vi "ECS-GDI-Host.vi"() -> ()   [LabVIEW 2015]
uses:
  <vilib>/addons/Software Calibration Management/XControls/SubHost.xctl
  <vilib>/addons/Software Calibration Management/XControls/SubHost List.xctl
  Typedefs/EPT/Engine Status.ctl
  <vilib>/addons/Software Calibration Management/XControls/TBL1D.xctl
  <vilib>/addons/Software Calibration Management/XControls/Faults.xctl
  ECS-Host.lvlib
  ECS-Shared.lvlib
panel:
  out "CalPointData":sgl[](array[numeric])
  in  "_Refresh":bool
  in  "EngineSpeed_MaxNC":sgl
  in  "EngineSpeed_MaxCrit":sgl
  out "5VPSU_CriticalFault":bool
  out "12VPSU_CriticalFault":bool
  out "BattV_CriticalFault":bool
  in  "_Main Tabs":T1(tab)
  in  "PowerEnable":bool caption="Power Enable"
  out "EngineSpeedFPGA1":sgl(knob) scale=0.0..1000.0 scale format="%#_6p"
  in  "SyncEnable":bool caption="Sync Enable"
  out "ReceivingPrimaryFPGA1":bool caption="Rcvg Primary"
  out "SyncFPGA1":bool caption="Sync"
  out "_BattVPresent":bool caption="Battery"
  out "_12VPresent":bool caption="12V"
  out "_5VPresent":bool caption="5V"
  out "Engine Time":sgl caption="[hr]" format="%0#5_4f"
  out "Time Since Start":sgl caption="[sec]" format="%05.0f"
  in  "Engine Time Reset":bool
  out "_Engine Speed":sgl format="%#.0f"
  out "Software Version":string caption="Version:"
  out "_Engine Status":T2 caption="Engine Status"
  in  "Faults Table":T4(xcontrol)
  in  "_SubHost Tab":T5(tab)
  in  "XNET CAN":T6(xcontrol)
  in  "Power":T6(xcontrol)
  in  "TDK High Voltage Supply":T6(xcontrol)
  in  "NI 9754-1 (ESTTL)":T6(xcontrol)
  in  "NI 9411-1 (Digital Input)":T6(xcontrol)
  in  "NI 9758-2 (PFI/LS)":T6(xcontrol)
  in  "NI 9751-4 (DI Driver)":T6(xcontrol)
  in  "NI 9751-3 (DI Driver)":T6(xcontrol)
  in  "NI 9751-2 (DI Driver)":T6(xcontrol)
  in  "NI 9752-1 (ADCombo)":T6(xcontrol)
  in  "NI 9757-1 (O2)":T6(xcontrol)
  in  "NI 9755-1 (NOx)":T6(xcontrol)
  in  "NI 9759-1 (Throttle)":T6(xcontrol)
  in  "NI 9758-1 (PFI/LS)":T6(xcontrol)
  in  "NI 9751-1 (DI Driver)":T6(xcontrol)
  in  "EPTx":T6(xcontrol)
  in  "Boost Actuation":T6(xcontrol)
  in  "Boost Actuation":T6(xcontrol)
  in  "MPCR":T6(xcontrol)
  in  "VVA Actuation":T6(xcontrol)
  in  "Direct Injectors":T6(xcontrol)
  in  "Engine Specs":T6(xcontrol)
  in  "Sensors":T6(xcontrol)
  in  "Faults":T6(xcontrol) caption="0"
  in  "Rail Pressure Setpoint":T6(xcontrol) caption="1"
  in  "Wastegate Control":T6(xcontrol) caption="1"
  in  "Turbo BPV Control":T6(xcontrol) caption="1"
  in  "Throttle Setpoint":T6(xcontrol) caption="1"
  in  "VVA Setpoint":T6(xcontrol) caption="1"
  in  "Intake Air Desired MAP":T6(xcontrol) caption="0"
  in  "Lambda Command":T6(xcontrol) caption="0"
  in  "Spark Control":T6(xcontrol) caption="1"
  in  "Cranking":T6(xcontrol) caption="0"
  in  "Direct Injection Strategy":T6(xcontrol) caption="2"
  in  "Fuel Quantity":T6(xcontrol) caption="1"
  in  "Load Command":T6(xcontrol) caption="0"
  in  "Intake Air Measured":T6(xcontrol) caption="1"
  in  "Execution Info":T6(xcontrol)
  in  "Calscope and Trends":T6(xcontrol)
  in  "MAP_ManE":bool
  in  "Pedal_ManE":bool
  in  "MEP_ManE":bool
  in  "RailP_ManE":bool
  in  "Pedal_Man":sgl(slide) caption="[bar]" scale=0.0..100.0 scale format="%#4.1f"
  in  "MEP_Man":sgl(slide) caption="[bar]" scale=0.0..25.0 scale format="%#4.1f"
  in  "RailP_Man":sgl(slide) caption="[bar]" scale=0.0..2000.0 scale format="%#4.1f"
  in  "MAP_Man":sgl(slide) caption="[kPa]" scale=0.0..400.0 scale format="%#4.1f"
  in  "ForceSafeState":bool caption="Push to Force Safe State"
  out "Non-Critical Fault":bool
  out "Critical Fault":bool
  in  "ESTOP":bool caption="Push to Stop"
  in  "System":T7(xcontrol)
  in  "Control":T7(xcontrol)
  in  "Engine":T7(xcontrol)
  in  "Hardware":T7(xcontrol)
  in  "_HiddenControls":enum32{"Page 1"}(tab)
  out "RailP_Des":sgl
  out "MAP_Des":sgl
  in  "NominalMEP_Tbl":cluster{"X":sgl[], "Y":sgl[]}(xcontrol)
  out "MEP_Des":sgl caption="EngineLoad_Des"
  out "Pedal_Des":sgl
  out "EngineStatus":u8
  in  "_Default Colors":bool caption="Default Colors"
  in  "_HiddenControls2":enum32{"Page 1"}(tab)
  in  "_VisiblePlots":bool[](array[boolean])
  in  "N Items":u8
  in  "_Signal Units":string[](array[string])
  in  "Colors":sgl[](array[numeric])
  in  "SliderMin":sgl[](array[numeric])
  in  "SliderMax":sgl[](array[numeric])
  out "Units":string
  in  "_Signal Names":string[](array[string])
  in  "CalPointIDs":sgl[](array[numeric])
  out "NamesLong":string
  out "_Chart":T8(graph)
  in  "_Down":bool
  in  "_Up":bool
  in  "_PlotHidden":bool caption="Hide"
  in  "_Delete":bool
  in  "_Add":bool
  out "_Data":string[](array[string])
  in  "_Slider Max":sgl caption="Max"
  in  "_Slider Min":sgl caption="Min"
  in  "_CalpointIDSelect":u16(ring) caption="Signal Name"
  in  "_Color":u32(colorbox)=16777222 caption="Color"
  in  "_Table":i32(listbox)
  in  "_Chart History1":i32=20 caption="Chart History"
  out "_LoadTracking":cluster{"X Buffer":sgl[], "Y Buffer":sgl[]}[](graph) caption="Load Tracking"
  in  "_Chart History2":i32=20 caption="Chart History"
  in  "_Normalize":bool=TRUE caption="Normalize"
  in  "_Var Select":u16(ring) caption="Signal Selection"
  out "_ReturnMap":cluster{"X Buffer":sgl[], "Y Buffer":sgl[]}[](graph) caption="Return Map"
  # "Engine Control System"
  # "RPM"
  # "Customize UI Here"
  # "Customize UI Here"
  # "Customize UI Here"
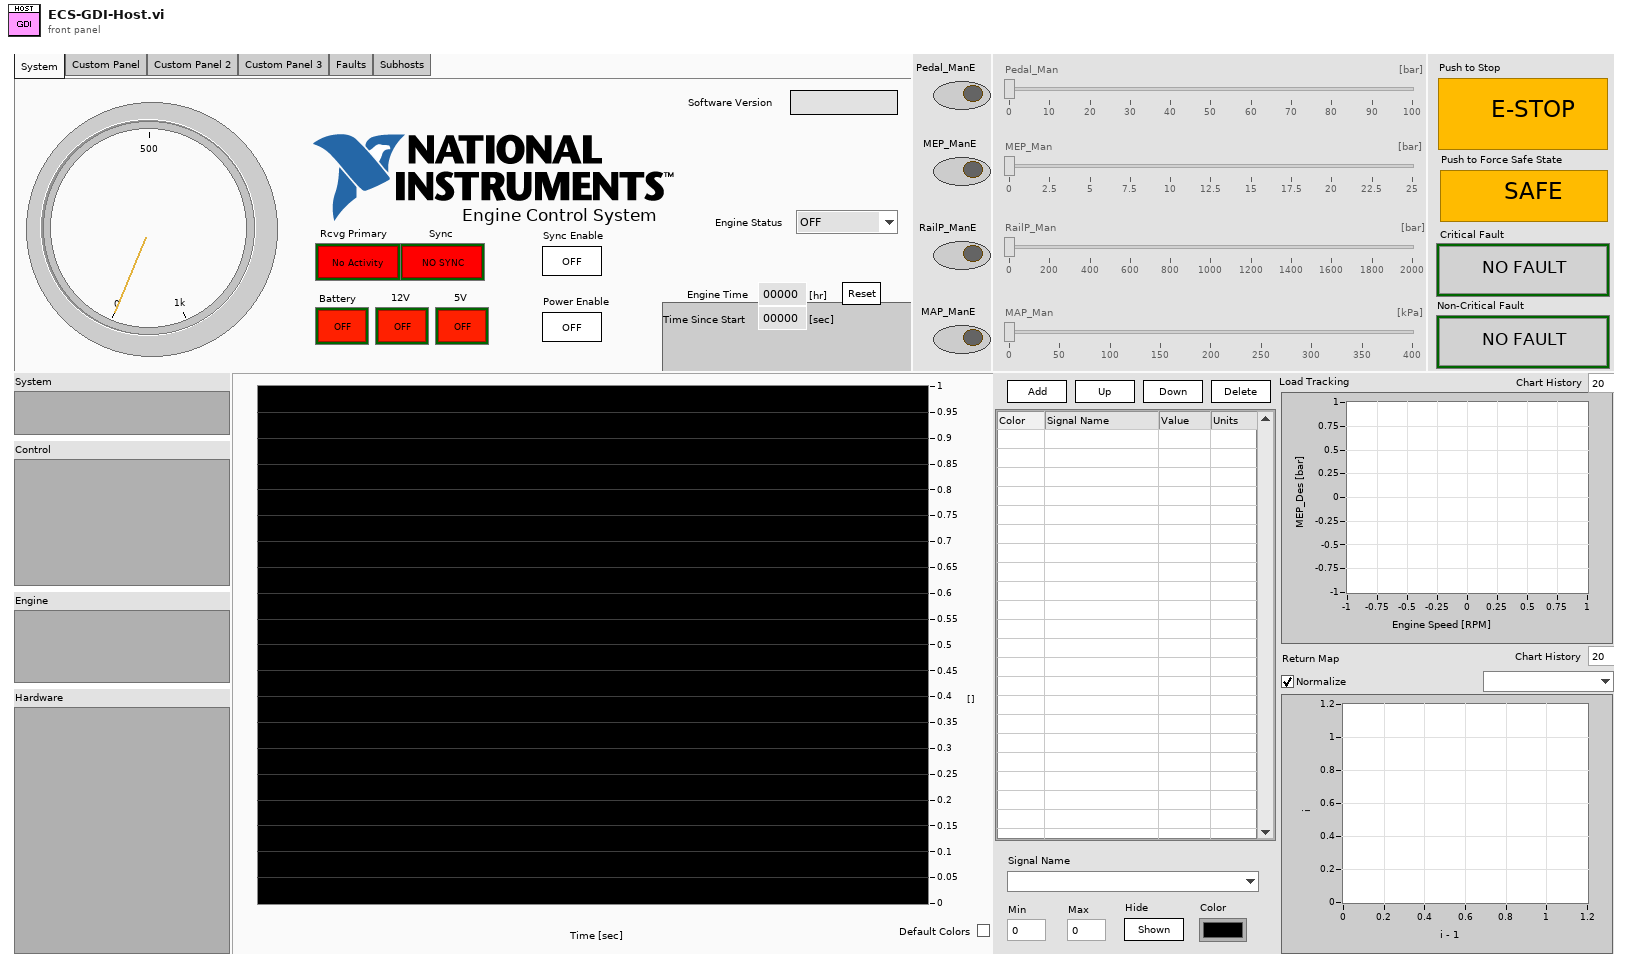
[diagram p1: front panel]
types:
  T1 = enum32{"System", "Custom Panel", "Custom Panel 2", "Custom Panel 3", "Faults", "Subhosts"}
  T2 = typedef "ECS-Shared.lvlib/Engine Status.ctl" = enum16{"OFF", "STALLED", "CRANKING", "RUNNING", "ACCEL", "DECEL", "SAFE"}
  T3 = typedef "Faults.xctl/Faults - Active.ctl" = cluster{"Highest Level":i32, "Very Low":u32, "Low":u32, "Medium":u32, "High":u32, "Very High":u32}
  T4 = cluster{"Active Faults":T3, "Unacknowledged Faults":T3}
  T5 = enum32{"Hardware I/O", "Engine I/O", "Control", "System"}
  T6 = cluster{"Name":string, "Host VI":path, "Pairing File":path, "Display Name":string}
  T7 = cluster{"States":enum32{"Invalid", "Standard", "Closed", "Hidden", "Minimized", "Maximized"}[], "VI Names":string[], "VI Refnums":refnum<vi>[], "Sub-Host Group":string, "Scrollbar":bool, "Listbox":refnum<vi>}
  T8 = cluster{"[0]":sgl, "[1]":sgl, "[2]":sgl, "[3]":sgl, "[4]":sgl, "[5]":sgl, "[6]":sgl, "[7]":sgl, "[8]":sgl, "[9]":sgl, "[10]":sgl, "[11]":sgl, "[12]":sgl, "[13]":sgl, "[14]":sgl, "[15]":sgl, "[16]":sgl, "[17]":sgl, "[18]":sgl, "[19]":sgl, "[20]":sgl, "[21]":sgl, "[22]":sgl, "[23]":sgl, "[24]":sgl, "[25]":sgl, "[26]":sgl, "[27]":sgl, "[28]":sgl, "[29]":sgl, "[30]":sgl, "[31]":sgl, "[32]":sgl, "[33]":sgl, "[34]":sgl, "[35]":sgl, "[36]":sgl, "[37]":sgl, "[38]":sgl, "[39]":sgl, "[40]":sgl, "[41]":sgl, "[42]":sgl, "[43]":sgl, "[44]":sgl, "[45]":sgl, "[46]":sgl, "[47]":sgl, "[48]":sgl, "[49]":sgl, "[50]":sgl, "[51]":sgl, "[52]":sgl, "[53]":sgl, "[54]":sgl, "[55]":sgl, "[56]":sgl, "[57]":sgl, "[58]":sgl, "[59]":sgl, "[60]":sgl, "[61]":sgl, "[62]":sgl, "[63]":sgl, "[64]":sgl, "[65]":sgl, "[66]":sgl, "[67]":sgl, "[68]":sgl, "[69]":sgl, "[70]":sgl, "[71]":sgl, "[72]":sgl, "[73]":sgl, "[74]":sgl, "[75]":sgl, "[76]":sgl, "[77]":sgl, "[78]":sgl, "[79]":sgl, "[80]":sgl, "[81]":sgl, "[82]":sgl, "[83]":sgl, "[84]":sgl, "[85]":sgl, "[86]":sgl, "[87]":sgl, "[88]":sgl, "[89]":sgl, "[90]":sgl, "[91]":sgl, "[92]":sgl, "[93]":sgl, "[94]":sgl, "[95]":sgl, "[96]":sgl, "[97]":sgl, "[98]":sgl, "[99]":sgl}
  T9 = enum8{"Enabled", "Disabled", "Disabled and Grayed Out"}
  T10 = cluster{"[0]":sgl, "[1]":sgl, "[2]":sgl, "[3]":sgl, "[4]":sgl, "[5]":sgl, "[6]":sgl, "[7]":sgl, "[8]":sgl, "[9]":sgl, "[10]":sgl, "[11]":sgl, "[12]":sgl, "[13]":sgl, "[14]":sgl, "[15]":sgl, "[16]":sgl, "[17]":sgl, "[18]":sgl, "[19]":sgl, "[20]":sgl, "[21]":sgl, "[22]":sgl, "[23]":sgl, "[24]":sgl, "[25]":sgl, "[26]":sgl, "[27]":sgl, "[28]":sgl, "[29]":sgl, "[30]":sgl, "[31]":sgl, "[32]":sgl, "[33]":sgl, "[34]":sgl, "[35]":sgl, "[36]":sgl, "[37]":sgl, "[38]":sgl, "[39]":sgl, "[40]":sgl, "[41]":sgl, "[42]":sgl, "[43]":sgl, "[44]":sgl, "[45]":sgl, "[46]":sgl, "[47]":sgl, "[48]":sgl, "[49]":sgl, "[50]":sgl, "[51]":sgl, "[52]":sgl, "[53]":sgl, "[54]":sgl, "[55]":sgl, "[56]":sgl, "[57]":sgl, "[58]":sgl, "[59]":sgl, "[60]":sgl, "[61]":sgl, "[62]":sgl, "[63]":sgl, "[64]":sgl, "[65]":sgl, "[66]":sgl, "[67]":sgl, "[68]":sgl, "[69]":sgl, "[70]":sgl, "[71]":sgl, "[72]":sgl, "[73]":sgl, "[74]":sgl, "[75]":sgl, "[76]":sgl, "[77]":sgl, "[78]":sgl, "[79]":sgl, "[80]":sgl, "[81]":sgl, "[82]":sgl, "[83]":sgl, "[84]":sgl, "[85]":sgl, "[86]":sgl, "[87]":sgl, "[88]":sgl, "[89]":sgl, "[90]":sgl, "[91]":sgl, "[92]":sgl, "[93]":sgl, "[94]":sgl, "[95]":sgl, "[96]":sgl, "[97]":sgl, "[98]":sgl, "[99]":sgl}[]
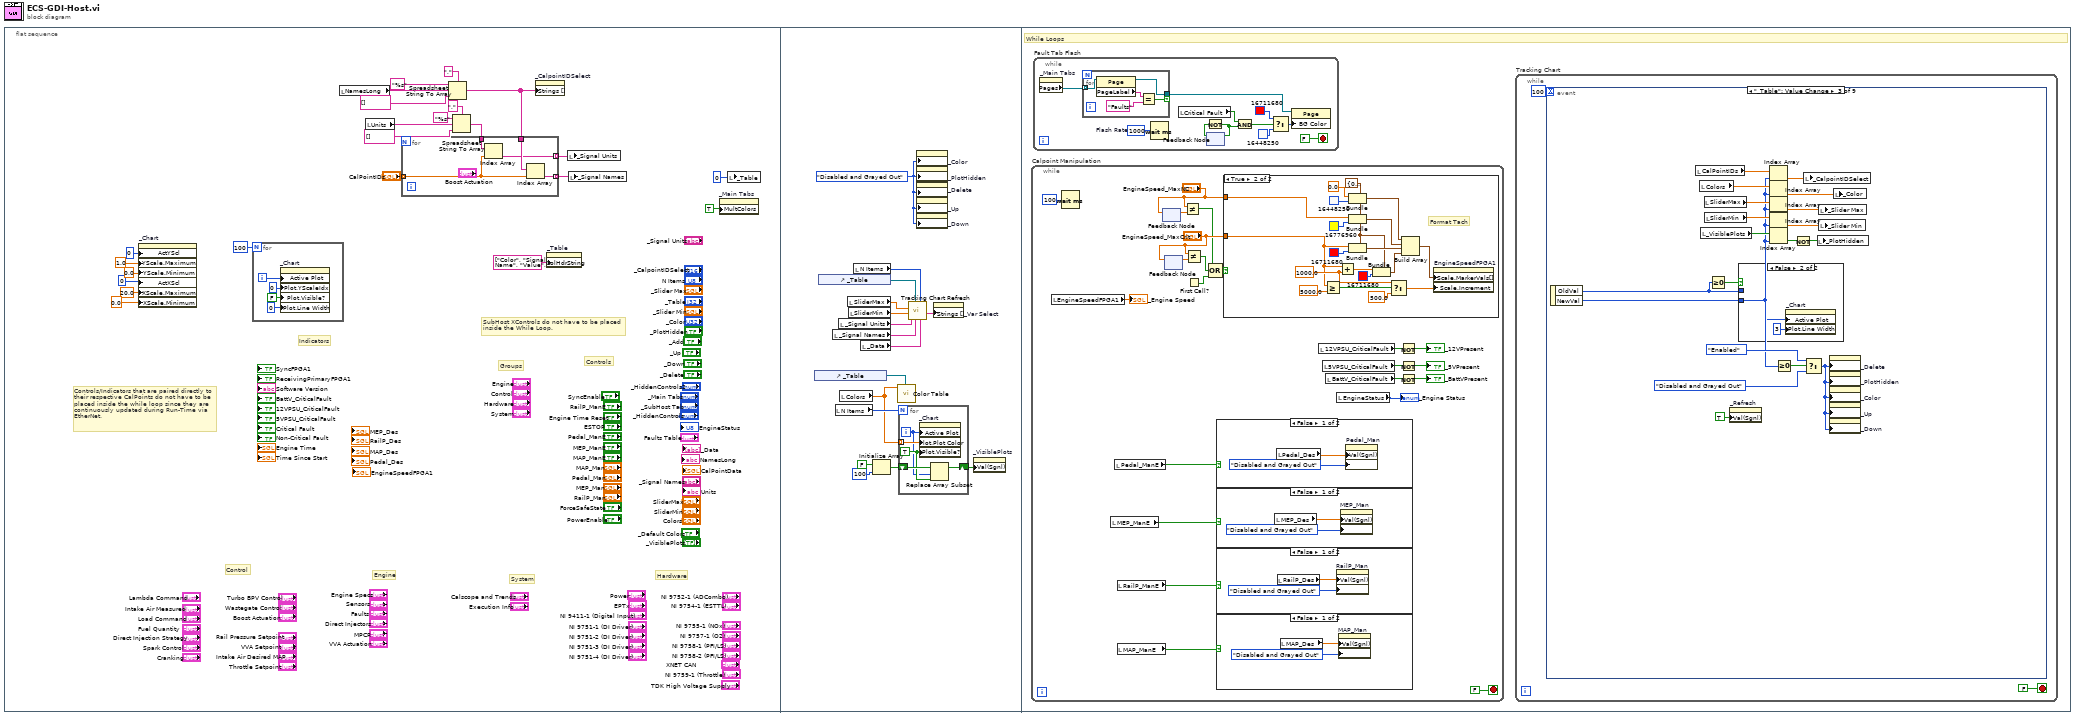
[diagram p0: block diagram]
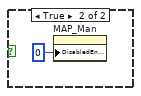
[diagram p2: hidden frame]
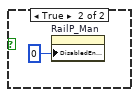
[diagram p3: hidden frame]
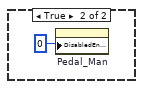
[diagram p4: hidden frame]
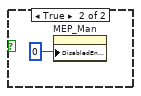
[diagram p5: hidden frame]
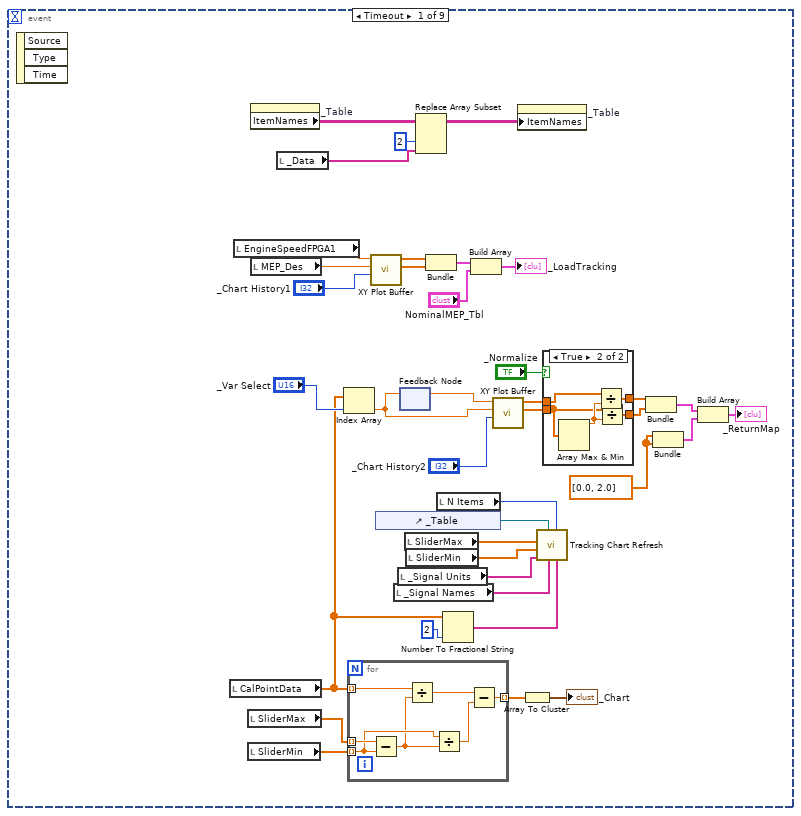
[diagram p7: hidden frame]
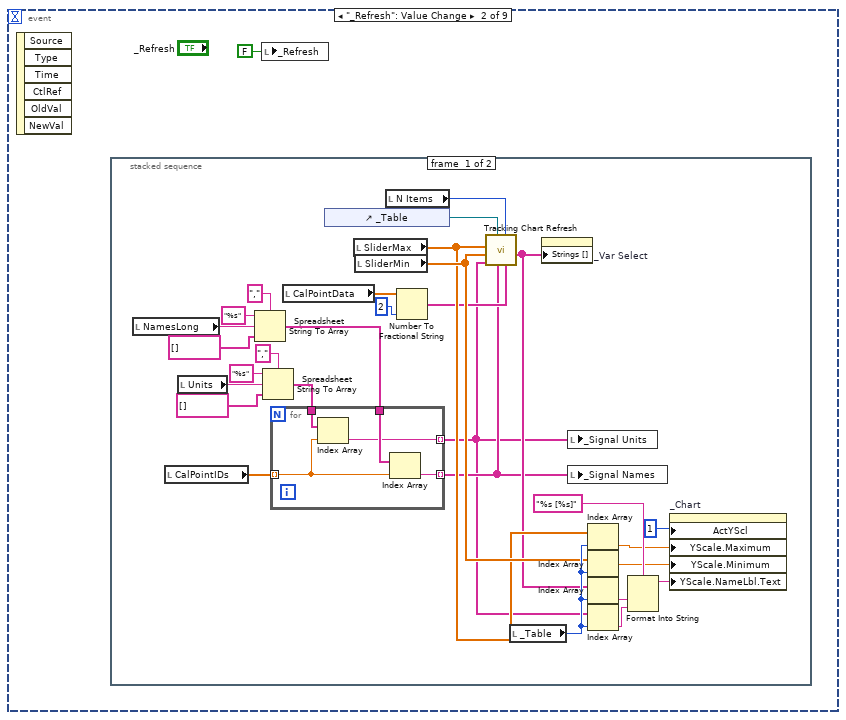
[diagram p9: hidden frame]
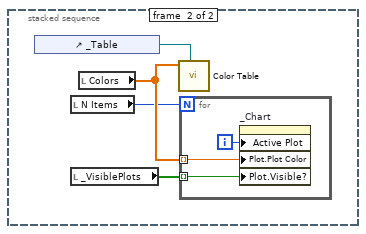
[diagram p10: hidden frame]
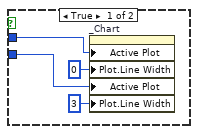
[diagram p11: hidden frame]
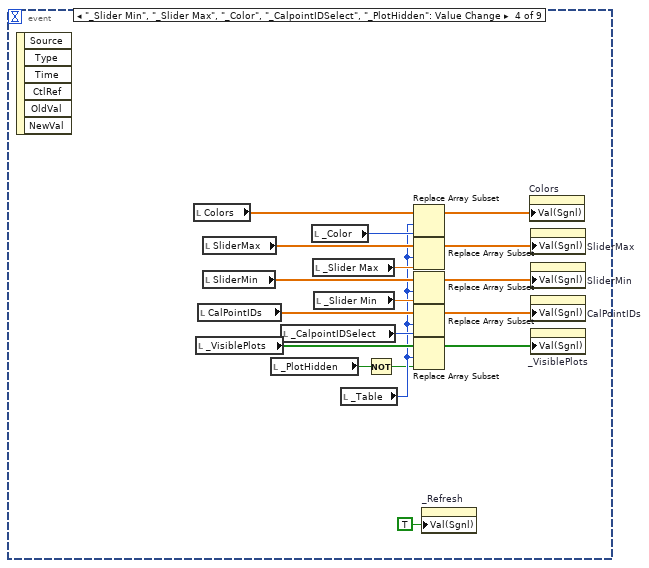
[diagram p12: hidden frame]
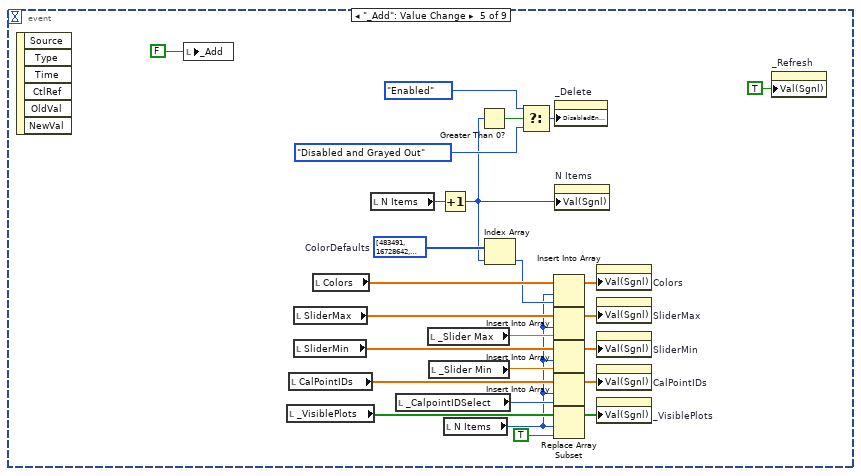
[diagram p13: hidden frame]
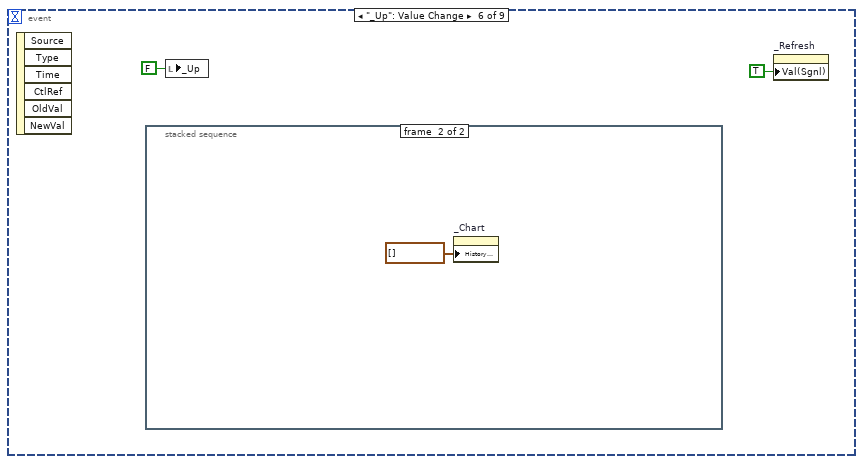
[diagram p14: hidden frame]
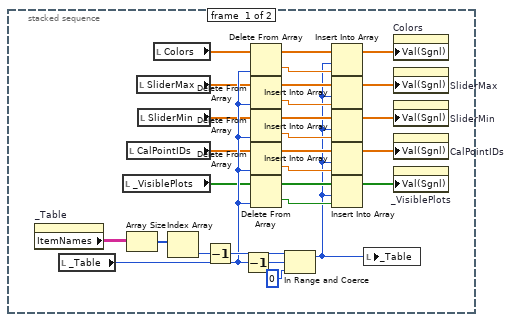
[diagram p15: hidden frame]
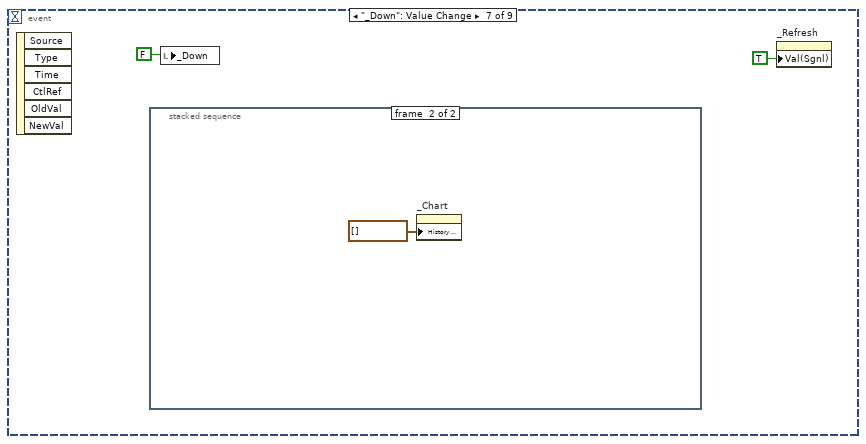
[diagram p16: hidden frame]
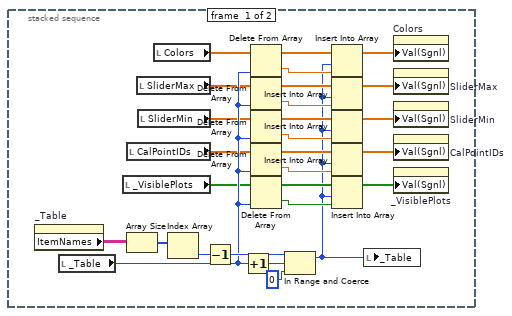
[diagram p17: hidden frame]
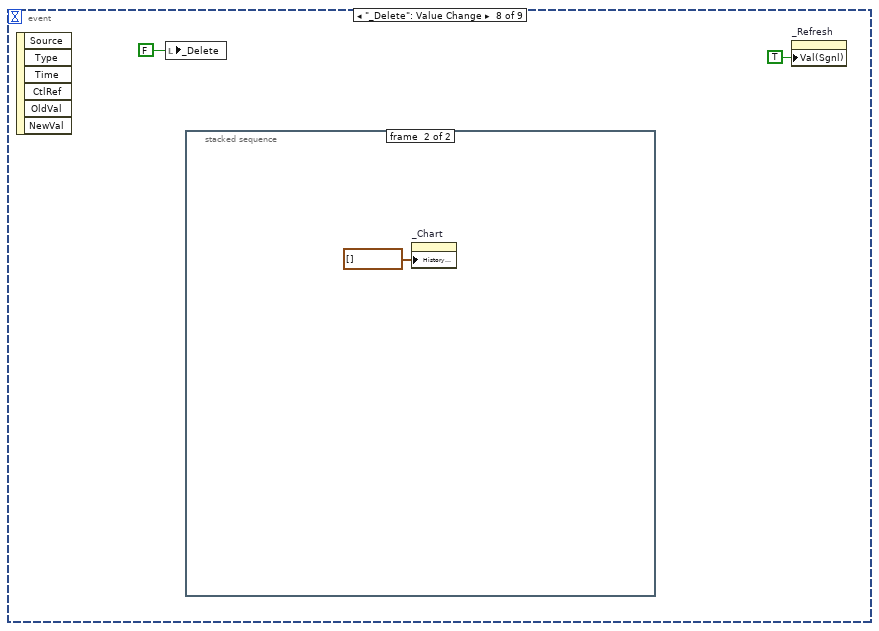
[diagram p18: hidden frame]
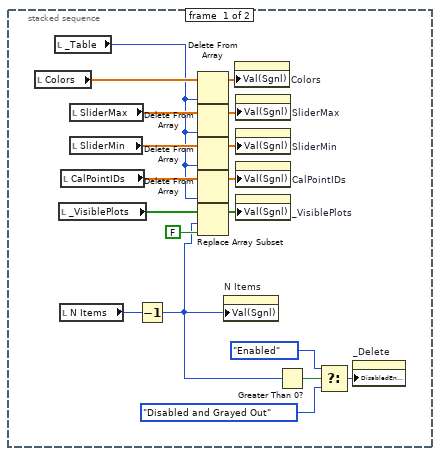
[diagram p19: hidden frame]
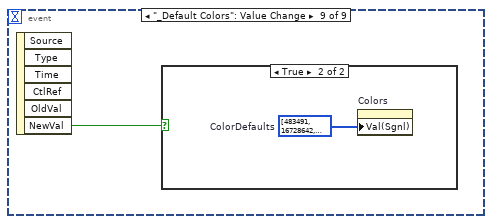
[diagram p20: hidden frame]
diagram:
  n1 = flat-sequence {
    frame #0 {
      # "System"
      # "Hardware"
      # "Engine"
      # "Control"
      # "Controls"
      # "Indicators"
      # "Groups"
      # "Controls/Indicators that are paired directly to their respective CalPoints do not have to be placed inside the while loop since they are continuously updated during Run-Time via EtherNet."
      # "SubHost XControls do not have to be placed inside the While Loop."
      n2 = property on="_Chart" class="WFChart (strict)"("ActYScl"=0 ("Active Y Scale"), "YScale.Maximum"=1.0 ("Y Scale.Range:Maximum"), "YScale.Minimum"=0.0 ("Y Scale.Range:Minimum"), "ActXScl"=0 ("Active X Scale"), "XScale.Maximum"=20.0 ("X Scale.Range:Maximum"), "XScale.Minimum"=0.0 ("X Scale.Range:Minimum")) -> ()  [unwired: 2 in, 2 out]
      n3 = for {
        N: 100 -> [_]
        i -> [w32]
        n4 = property on="_Chart" class="WFChart (strict)"("Active Plot"=w32, "Plot.YScaleIdx"=u32 0 ("Plot.Y Scale Index"), "Plot.Visible?"=FALSE ("Plot.Visible"), "Plot.Line Width"=u8 0) -> ()  [unwired: 2 in, 2 out]
      }
      n5 = local read "NamesLong"() -> (w11:string)
      n6 = local read "Units"() -> (w7:string)
      n7 = Spreadsheet String To Array(delimiter (Tab)=",", format string="%s", spreadsheet string=w11, array type (2D Dbl)=string[] []) -> (array=w3:string[])
      n8 = Spreadsheet String To Array(delimiter (Tab)=",", format string="%s", spreadsheet string=w7, array type (2D Dbl)=string[] []) -> (array=w6:string[])
      n9 = for {
        tunnel: "CalPointIDs" -> [w25] mode=indexing
        tunnel: w3 -> [w28]
        tunnel: [w27] -> w4 mode=indexing
        tunnel: w6 -> [w26]
        tunnel: [w24] -> w2 mode=indexing
        n10 = Index Array(array=w26, index=w25) -> (element=w24:string)
        n11 = Index Array(array=w28, index=w25) -> (element=w27:string)
      }
      n12 = property on="_CalpointIDSelect" class="Ring (strict)"("Strings []"=w3) -> ()  [unwired: 2 in, 2 out]
      n13 = property on="_Table" class="MCListbox (strict)"("ColHdrString"=string[] ["Color", "Signal Name", "Value", "Units"] ("Column Header Strings[]")) -> ()  [unwired: 2 in, 2 out]
      n14 = local write "_Signal Units"(w2) -> ()
      n15 = local write "_Signal Names"(w4) -> ()
      n16 = property on="_Main Tabs" class="TabCtl (strict)"("MultColors"=TRUE ("Allow Multiple Colors")) -> ()  [unwired: 2 in, 2 out]
      n17 = local write "_Table"(0 ("Value (Signaling)")) -> ()
    }
    frame #1 {
      w33 = T9."Disabled and Grayed Out" ("Disabled")
      n18 = control-ref of="_Table"() -> (w38:refnum<vi>)
      n19 = control-ref of="_Table"() -> (w48:refnum<vi>)
      n20 = local read "_Signal Names"() -> (w46:string[])
      n21 = local read "N Items"() -> (w40:u8)
      n22 = local read "_Signal Units"() -> (w43:string[])
      n23 = local read "Colors"() -> (w39:sgl[])
      n24 = local read "SliderMax"() -> (w45:sgl[])
      n25 = local read "SliderMin"() -> (w44:sgl[])
      n26 = local read "N Items"() -> (w42:u8)
      n27 = local read "_Data"() -> (w47:string[])
      n28 = Initialize Array(FALSE, 100 ("dimension size")) -> (w35:bool[])
      n29 = call "Color Table.vi"("_Table"=w38, "Colors"=w39) -> ()  [unwired: 10 in]
      n30 = for {
        N: w40 -> [_]
        tunnel: w39 -> [w53] mode=indexing
        shift-right: [w51] -> w34
        shift-left: w35 -> [w52]
        i -> [w49]
        w50 = TRUE ("Plot.Visible")
        n31 = property on="_Chart" class="WFChart (strict)"("Active Plot"=w49, "Plot.Plot Color"=w53, "Plot.Visible?"=w50) -> ()  [unwired: 2 in, 2 out]
        n32 = Replace Array Subset(array=w52, new element=w50, index=w49) -> (w51:bool[])
      }
      n33 = call "Tracking Chart Refresh.vi"("Data"=w47, "N Items"=w42, "Signal Names"=w46, "_Table"=w48, "Signal Units"=w43, "Slider Min"=w44, "Slider Max"=w45) -> ("Short Signal Names"=w41:string[])  [unwired: 4 in]
      n34 = property on="_Color" class="ColBox"("DisabledEnum"=w33) -> ()  [unwired: 2 in, 2 out]
      n35 = property on="_PlotHidden" class="Bool (strict)"("DisabledEnum"=w33) -> ()  [unwired: 2 in, 2 out]
      n36 = property on="_Delete" class="Bool (strict)"("DisabledEnum"=w33) -> ()  [unwired: 2 in, 2 out]
      n37 = property on="_Up" class="Bool (strict)"("DisabledEnum"=w33) -> ()  [unwired: 2 in, 2 out]
      n38 = property on="_Down" class="Bool (strict)"("DisabledEnum"=w33) -> ()  [unwired: 2 in, 2 out]
      n39 = property on="_Var Select" class="Ring (strict)"("Strings []"=w41) -> ()  [unwired: 2 in, 2 out]
      n40 = property on="_VisiblePlots" class="Arr (strict)"("Val(Sgnl)"=w34) -> ()  [unwired: 2 in, 2 out]
    }
    frame #2 {
      # "While Loops"
      n41 = while "Calpoint Manipulation" {
        stop <- FALSE stop-if-true
        n42 = local read "EngineSpeedFPGA1"() -> (→"_Engine Speed":sgl)
        n43 = Wait (ms)(milliseconds to wait=u32 100) -> ()  [unwired: 1 out]
        n44 = local read "MEP_ManE"() -> (w74:bool)
        n45 = local read "Pedal_ManE"() -> (w73:bool)
        n46 = local read "RailP_ManE"() -> (w72:bool)
        n47 = local read "MAP_ManE"() -> (w71:bool)
        n48 = feedback #1() -> (w80:sgl)  [unwired: 1 in]
        n49 = feedback-in #1("EngineSpeed_MaxNC") -> ()
        n50 = feedback #2() -> (w88:sgl)  [unwired: 1 in]
        n51 = feedback-in #2("EngineSpeed_MaxCrit") -> ()
        n52 = Not Equal?(x="EngineSpeed_MaxNC", y=w80) -> (x != y?=w77:bool)
        n53 = Not Equal?(x="EngineSpeed_MaxCrit", y=w88) -> (x != y?=w76:bool)
        n54 = First Call?() -> (First Call?: T/F=w78:bool)
        n55 = Compound Arithmetic op=OR(w77, w76, w78) -> (w79:bool)
        n56 = case shown="False" w73 {
          frame False {
            n57 = local read "Pedal_Des"() -> (w98:sgl)
            n58 = property on="Pedal_Man" class="Slide (strict)"("Val(Sgnl)"=w98, "DisabledEnum"=T9."Disabled and Grayed Out" ("Disabled")) -> ()  [unwired: 2 in, 2 out]
          }
          frame True {
            n59 = property on="Pedal_Man" class="Slide (strict)"("DisabledEnum"=u8 0) -> ()  [unwired: 2 in, 2 out]
          }
        }
        n60 = case shown="False" w74 {
          frame False {
            n61 = local read "MEP_Des"() -> (w102:sgl)
            n62 = property on="MEP_Man" class="Slide (strict)"("Val(Sgnl)"=w102, "DisabledEnum"=T9."Disabled and Grayed Out" ("Disabled")) -> ()  [unwired: 2 in, 2 out]
          }
          frame True {
            n63 = property on="MEP_Man" class="Slide (strict)"("DisabledEnum"=u8 0) -> ()  [unwired: 2 in, 2 out]
          }
        }
        n64 = case shown="False" w72 {
          frame False {
            n65 = local read "RailP_Des"() -> (w95:sgl)
            n66 = property on="RailP_Man" class="Slide (strict)"("Val(Sgnl)"=w95, "DisabledEnum"=T9."Disabled and Grayed Out" ("Disabled")) -> ()  [unwired: 2 in, 2 out]
          }
          frame True {
            n67 = property on="RailP_Man" class="Slide (strict)"("DisabledEnum"=u8 0) -> ()  [unwired: 2 in, 2 out]
          }
        }
        n68 = case shown="False" w71 {
          frame False {
            n69 = local read "MAP_Des"() -> (w92:sgl)
            n70 = property on="MAP_Man" class="Slide (strict)"("Val(Sgnl)"=w92, "DisabledEnum"=T9."Disabled and Grayed Out" ("Disabled")) -> ()  [unwired: 2 in, 2 out]
          }
          frame True {
            n71 = property on="MAP_Man" class="Slide (strict)"("DisabledEnum"=u8 0) -> ()  [unwired: 2 in, 2 out]
          }
        }
        n72 = case shown="True" w79 {
          tunnel: "EngineSpeed_MaxCrit" -> [_ w111]
          tunnel: "EngineSpeed_MaxNC" -> [_ w105]
          frame False {
          }
          frame True {
            w112 = sgl 1000.0 ("y")
            w108 = cluster{dbl, u32} {0.0, 0}
            # "Format Tach"
            n73 = Greater Or Equal?(x=w111, y=sgl 5000.0) -> (x >= y?=w114:bool)
            n74 = Add(x=w111, y=w112) -> (x+y=w116:sgl)
            n75 = Bundle(cluster=w108, sgl 0.0, u32 16448250) -> (w107:cluster{dbl, u32})
            n76 = Bundle(cluster=w108, w105, u32 16776960) -> (w106:cluster{dbl, u32})
            n77 = Bundle(cluster=w108, w111, u32 16711680) -> (w122:cluster{dbl, u32})
            n78 = Bundle(cluster=w108, w116, u32 16711680) -> (w119:cluster{dbl, u32})
            n79 = Select(t=w112, s=w114, f=sgl 500.0 ("Scale.Range:Increment")) -> (s? t:f=w109:sgl)
            n80 = Build Array(w107, w106, w122, w119) -> (w110:cluster{dbl, u32}[])
            n81 = property on="EngineSpeedFPGA1" class="Knob (strict)"("Scale.MarkerVals[]"=w110, "Scale.Increment"=w109) -> ()  [unwired: 2 in, 2 out]
          }
        }
        n82 = local read "12VPSU_CriticalFault"() -> (w84:bool)
        n83 = local read "5VPSU_CriticalFault"() -> (w85:bool)
        n84 = local read "BattV_CriticalFault"() -> (w86:bool)
        n85 = local read "EngineStatus"() -> (→"_Engine Status":u8)
        n86 = Not(x=w84) -> (.not. x?=→"_12VPresent":bool)
        n87 = Not(x=w85) -> (.not. x?=→"_5VPresent":bool)
        n88 = Not(x=w86) -> (.not. x?=→"_BattVPresent":bool)
      }
      n89 = while "Fault Tab Flash" {
        stop <- FALSE stop-if-true
        w63 = u32 1000  # Flash Rate
        n90 = property on="_Main Tabs" class="TabCtl (strict)"() -> ("Pages"=w55:refnum<vi>[])  [unwired: 2 in, 2 out]
        n91 = for {
          tunnel: w55 -> [w69] mode=indexing
          tunnel: [w65] -> w54 if=w66
          n92 = property class="Page"(reference=w69) -> (reference out=w65:refnum<vi>, "PageLabel"=w68:string)  [unwired: 1 in, 1 out]
          n93 = Equal?(x=w68, y="Faults") -> (x = y?=w66:bool)
        }
        n94 = Wait (ms)(milliseconds to wait=w63) -> ()  [unwired: 1 out]
        n95 = local read "Critical Fault"() -> (w56:bool)
        n96 = feedback #3() -> (w60:bool)  [unwired: 1 in]
        n97 = Not(x=w60) -> (.not. x?=w61:bool)
        n98 = feedback-in #3(w61) -> ()
        n99 = And(x=w56, y=w61) -> (x .and. y?=w59:bool)
        n100 = Select(t=u32 16711680, s=w59, f=u32 16448250) -> (s? t:f=w58:u32)
        n101 = property class="Page"(reference=w54, "BG Color"=w58) -> ()  [unwired: 1 in, 2 out]
      }
      n102 = while "Tracking Chart" {
        stop <- FALSE stop-if-true
        n103 = event shown="[2] \"_Table\": Value Change" {
          selector: _ -> [_ _ _ _ _ _ _ _ _]
          dyn-events: _ -> [_ _ _ _ _ _ _ _ _]
          timeout: 100 -> [_ _ _ _ _ _ _ _ _]
          event Timeout {
            w145 = sgl[] [0.0, 2.0]
            n104 = event-data() -> ()  [unwired: 1 in, 3 out]
            n105 = local read "CalPointData"() -> (w134:sgl[])
            n106 = local read "EngineSpeedFPGA1"() -> (w152:sgl)
            n107 = local read "SliderMax"() -> (w133:sgl[])
            n108 = local read "SliderMin"() -> (w132:sgl[])
            n109 = property on="_Table" class="MCListbox (strict)"() -> ("ItemNames"=w162:string[][])  [unwired: 2 in, 2 out]
            n110 = local read "MEP_Des"() -> (w151:sgl)
            n111 = local read "_Data"() -> (w161:string[])
            n112 = Index Array(array=w134, index="_Var Select") -> (element=w150:sgl)
            n113 = for {
              tunnel: w134 -> [w166] mode=indexing
              tunnel: [w163] -> w135 mode=indexing
              tunnel: w133 -> [w168] mode=indexing
              tunnel: w132 -> [w167] mode=indexing
              n114 = Subtract(x=w168, y=w167) -> (x-y=w165:sgl)
              n115 = Divide(x=w166, y=w165) -> (x/y=w169:sgl)
              n116 = Divide(x=w167, y=w165) -> (x/y=w164:sgl)
              n117 = Subtract(x=w169, y=w164) -> (x-y=w163:sgl)
            }
            n118 = call "XY Plot Buffer.vi"("History Length"="_Chart History1", "Input 2"=w151, "Input 1"=w152) -> ("Y Buffer"=w154:sgl[], "X Buffer"=w155:sgl[])  [unwired: 7 in]
            n119 = control-ref of="_Table"() -> (w131:refnum<vi>)
            n120 = local read "_Signal Names"() -> (w126:string[])
            n121 = local read "_Signal Units"() -> (w125:string[])
            n122 = feedback #4() -> (w149:sgl)  [unwired: 1 in]
            n123 = feedback-in #4(w150) -> ()
            n124 = local read "SliderMax"() -> (w128:sgl[])
            n125 = local read "SliderMin"() -> (w129:sgl[])
            n126 = Replace Array Subset(array=w162, new element=w161, index (col)=2 ("disabled index (col)")) -> (w159:string[][])  [unwired: 1 in]
            n127 = Bundle("X Buffer"=w155, "Y Buffer"=w154) -> (w157:cluster{"X Buffer":sgl[], "Y Buffer":sgl[]})  [unwired: 1 in]
            n128 = local read "N Items"() -> (w130:u8)
            n129 = Number To Fractional String(number=w134, precision (6)=i16 2) -> (F-format string=w127:string[])  [unwired: 2 in]
            n130 = Build Array(w157, "NominalMEP_Tbl") -> (→"_LoadTracking":cluster{"X":sgl[], "Y":sgl[]}[])
            n131 = call "XY Plot Buffer.vi"("History Length"="_Chart History2", "Input 2"=w150, "Input 1"=w149) -> ("Y Buffer"=w141:sgl[], "X Buffer"=w139:sgl[])  [unwired: 7 in]
            n132 = property on="_Table" class="MCListbox (strict)"("ItemNames"=w159) -> ()  [unwired: 2 in, 2 out]
            n133 = Array To Cluster(array=w135) -> (cluster=→"_Chart":T8)
            n134 = call "Tracking Chart Refresh.vi"("Data"=w127, "N Items"=w130, "Signal Names"=w126, "_Table"=w131, "Signal Units"=w125, "Slider Min"=w129, "Slider Max"=w128) -> ()  [unwired: 4 in, 1 out]
            n135 = case shown="True" "_Normalize" {
              tunnel: [w171 w176] -> w138
              tunnel: w139 -> [w171 w175]
              tunnel: [w170 w173] -> w140
              tunnel: w141 -> [w170 w172]
              frame False {
              }
              frame True {
                n136 = Array Max & Min(array=w172) -> (max value=w174:sgl)  [unwired: 3 out]
                n137 = Divide(x=w175, y=w174) -> (x/y=w176:sgl[])
                n138 = Divide(x=w172, y=w174) -> (x/y=w173:sgl[])
              }
            }
            n139 = Bundle("X Buffer"=w138, "Y Buffer"=w140) -> (w146:cluster{"X Buffer":sgl[], "Y Buffer":sgl[]})  [unwired: 1 in]
            n140 = Bundle(w145, w145) -> (w147:cluster{sgl[], sgl[]})  [unwired: 1 in]
            n141 = Build Array(w146, w147) -> (→"_ReturnMap":cluster{"X Buffer":sgl[], "Y Buffer":sgl[]}[])
          }
          event "_Refresh": Value Change {
            n142 = event-data() -> ()  [unwired: 1 in, 6 out]
            n143 = stacked-sequence {
              frame #0 {
                n144 = local read "NamesLong"() -> (w202:string)
                n145 = local read "CalPointIDs"() -> (w200:sgl[])
                n146 = local read "Units"() -> (w194:string)
                n147 = Spreadsheet String To Array(delimiter (Tab)=",", format string="%s", spreadsheet string=w202, array type (2D Dbl)=string[] []) -> (array=w201:string[])
                n148 = Spreadsheet String To Array(delimiter (Tab)=",", format string="%s", spreadsheet string=w194, array type (2D Dbl)=string[] []) -> (array=w187:string[])
                n149 = for {
                  tunnel: w200 -> [w208] mode=indexing
                  tunnel: w201 -> [w211]
                  tunnel: [w210] -> w179 mode=indexing
                  tunnel: w187 -> [w209]
                  tunnel: [w207] -> w178 mode=indexing
                  n150 = Index Array(array=w209, index=w208) -> (element=w207:string)
                  n151 = Index Array(array=w211, index=w208) -> (element=w210:string)
                }
                n152 = local read "CalPointData"() -> (w181:sgl[])
                n153 = control-ref of="_Table"() -> (w206:refnum<vi>)
                n154 = local read "SliderMax"() -> (w184:sgl[])
                n155 = local read "SliderMin"() -> (w185:sgl[])
                n156 = local read "N Items"() -> (w186:u8)
                n157 = Number To Fractional String(number=w181, precision (6)=i16 2) -> (F-format string=w180:string[])  [unwired: 2 in]
                n158 = call "Tracking Chart Refresh.vi"("Data"=w180, "N Items"=w186, "Signal Names"=w179, "_Table"=w206, "Signal Units"=w178, "Slider Min"=w185, "Slider Max"=w184) -> ("Short Signal Names"=w183:string[])  [unwired: 4 in]
                n159 = local read "_Table"() -> (w198:i32)
                n160 = property on="_Var Select" class="Ring (strict)"("Strings []"=w183) -> ()  [unwired: 2 in, 2 out]
                n161 = local write "_Signal Units"(w178) -> ()
                n162 = local write "_Signal Names"(w179) -> ()
                n163 = Index Array(array=w184, index=w198) -> (element=w190:sgl)
                n164 = Index Array(array=w185, index=w198) -> (element=w189:sgl)
                n165 = Index Array(array=w183, index=w198) -> (element=w188:string)
                n166 = Index Array(array=w178, index=w198) -> (element=w193:string)
                n167 = Format Into String(format string="%s [%s]", w188, w193) -> (resulting string=w191:string)  [unwired: 2 in, 1 out]
                n168 = property on="_Chart" class="WFChart (strict)"("ActYScl"=1 ("Active Y Scale"), "YScale.Maximum"=w190, "YScale.Minimum"=w189, "YScale.NameLbl.Text"=w191) -> ()  [unwired: 2 in, 2 out]
              }
              frame #1 {
                n169 = control-ref of="_Table"() -> (w215:refnum<vi>)
                n170 = local read "N Items"() -> (w213:u8)
                n171 = local read "_VisiblePlots"() -> (w212:bool[])
                n172 = local read "Colors"() -> (w214:sgl[])
                n173 = call "Color Table.vi"("_Table"=w215, "Colors"=w214) -> ()  [unwired: 10 in]
                n174 = for {
                  N: w213 -> [_]
                  tunnel: w214 -> [w217] mode=indexing
                  tunnel: w212 -> [w216] mode=indexing
                  i -> [w218]
                  n175 = property on="_Chart" class="WFChart (strict)"("Active Plot"=w218, "Plot.Plot Color"=w217, "Plot.Visible?"=w216) -> ()  [unwired: 2 in, 2 out]
                }
              }
            }
            n176 = local write "_Refresh"(FALSE ("_Refresh")) -> ()
          }
          event "_Table": Value Change {
            n177 = event-data() -> ("OldVal"=w219:i32, "NewVal"=w222:i32)  [unwired: 1 in]
            n178 = local read "CalPointIDs"() -> (w233:sgl[])
            n179 = local read "Colors"() -> (w237:sgl[])
            n180 = local read "_VisiblePlots"() -> (w227:bool[])
            n181 = local read "SliderMax"() -> (w236:sgl[])
            n182 = local read "SliderMin"() -> (w235:sgl[])
            n183 = Greater Or Equal To 0?(x=w219) -> (x >= 0?=w220:bool)
            n184 = property on="_Refresh" class="Bool (strict)"("Val(Sgnl)"=TRUE ("Value (Signaling)")) -> ()  [unwired: 2 in, 2 out]
            n185 = case shown="False" w220 {
              tunnel: w219 -> [w241 _]
              tunnel: w222 -> [w238 w242]
              frame True {
                n186 = property on="_Chart" class="WFChart (strict)"("Active Plot"=w241, "Plot.Line Width"=u8 0, "Active Plot"=w238, "Plot.Line Width"=u8 3) -> ()  [unwired: 2 in, 2 out]
              }
              frame False {
                n187 = property on="_Chart" class="WFChart (strict)"("Active Plot"=w242, "Plot.Line Width"=u8 3) -> ()  [unwired: 2 in, 2 out]
              }
            }
            n188 = Index Array(array=w233, index=w222) -> (element=w231:sgl)
            n189 = Index Array(array=w237, index=w222) -> (element=w234:sgl)
            n190 = Index Array(array=w236, index=w222) -> (element=w230:sgl)
            n191 = Index Array(array=w235, index=w222) -> (element=w229:sgl)
            n192 = Index Array(array=w227, index=w222) -> (element=w228:bool)
            n193 = Greater Or Equal To 0?(x=w222) -> (x >= 0?=w223:bool)
            n194 = Not(x=w228) -> (.not. x?=w226:bool)
            n195 = local write "_CalpointIDSelect"(w231) -> ()
            n196 = Select(t=T9."Enabled" ("Disabled"), s=w223, f=T9."Disabled and Grayed Out" ("Disabled")) -> (s? t:f=w221:T9)
            n197 = local write "_PlotHidden"(w226) -> ()
            n198 = local write "_Slider Max"(w230) -> ()
            n199 = local write "_Slider Min"(w229) -> ()
            n200 = property on="_Delete" class="Bool (strict)"("DisabledEnum"=w221) -> ()  [unwired: 2 in, 2 out]
            n201 = property on="_PlotHidden" class="Bool (strict)"("DisabledEnum"=w221) -> ()  [unwired: 2 in, 2 out]
            n202 = property on="_Color" class="ColBox"("DisabledEnum"=w221) -> ()  [unwired: 2 in, 2 out]
            n203 = property on="_Up" class="Bool (strict)"("DisabledEnum"=w221) -> ()  [unwired: 2 in, 2 out]
            n204 = property on="_Down" class="Bool (strict)"("DisabledEnum"=w221) -> ()  [unwired: 2 in, 2 out]
            n205 = local write "_Color"(w234) -> ()
          }
          event "_Slider Min", "_Slider Max", "_Color", "_CalpointIDSelect", "_PlotHidden": Value Change {
            n206 = event-data() -> ()  [unwired: 1 in, 6 out]
            n207 = local read "Colors"() -> (w257:sgl[])
            n208 = local read "_VisiblePlots"() -> (w248:bool[])
            n209 = local read "CalPointIDs"() -> (w250:sgl[])
            n210 = local read "SliderMax"() -> (w258:sgl[])
            n211 = local read "SliderMin"() -> (w261:sgl[])
            n212 = local read "_PlotHidden"() -> (w247:bool)
            n213 = local read "_CalpointIDSelect"() -> (w251:u16)
            n214 = local read "_Color"() -> (w256:u32)
            n215 = local read "_Slider Max"() -> (w259:sgl)
            n216 = local read "_Slider Min"() -> (w260:sgl)
            n217 = local read "_Table"() -> (w245:i32)
            n218 = Not(x=w247) -> (.not. x?=w244:bool)
            n219 = Replace Array Subset(array=w257, new element=w256, index=w245) -> (w249:sgl[])
            n220 = Replace Array Subset(array=w258, new element=w259, index=w245) -> (w255:sgl[])
            n221 = Replace Array Subset(array=w261, new element=w260, index=w245) -> (w254:sgl[])
            n222 = Replace Array Subset(array=w250, new element=w251, index=w245) -> (w252:sgl[])
            n223 = Replace Array Subset(array=w248, new element=w244, index=w245) -> (w246:bool[])
            n224 = property on="_Refresh" class="Bool (strict)"("Val(Sgnl)"=TRUE ("Value (Signaling)")) -> ()  [unwired: 2 in, 2 out]
            n225 = property on="Colors" class="Arr (strict)"("Val(Sgnl)"=w249) -> ()  [unwired: 2 in, 2 out]
            n226 = property on="SliderMax" class="Arr (strict)"("Val(Sgnl)"=w255) -> ()  [unwired: 2 in, 2 out]
            n227 = property on="SliderMin" class="Arr (strict)"("Val(Sgnl)"=w254) -> ()  [unwired: 2 in, 2 out]
            n228 = property on="CalPointIDs" class="Arr (strict)"("Val(Sgnl)"=w252) -> ()  [unwired: 2 in, 2 out]
            n229 = property on="_VisiblePlots" class="Arr (strict)"("Val(Sgnl)"=w246) -> ()  [unwired: 2 in, 2 out]
          }
          event "_Add": Value Change {
            w271 = u32[] [483491, 16728642, 982784, 4375295, 13827953, 13457919, 16757522, 4343295, 16728758, 5898228, 16448250, 16728642, 982784, 4375295, 13827953, 13457919, 16757522, 4343295, 16728758, 5898228, 16448250, 16728642, 982784, 4375295, 13827953, 13457919, 16757522, 4343295, 16728758, 5898228, 16448250, 16728642, 982784, 4375295, 13827953, 13457919, 16757522, 4343295, 16728758, 5898228, 16448250, 16728642, 982784, 4375295, 13827953, 13457919, 16757522, 4343295, 16728758, 5898228, 16448250, 16728642, 982784, 4375295, 13827953, 13457919, 16757522, 4343295, 16728758, 5898228, 16448250, 16728642, 982784, 4375295, 13827953, 13457919, 16757522, 4343295, 16728758, 5898228, 16448250, 16728642, 982784, 4375295, 13827953, 13457919, 16757522, 4343295, 16728758, 5898228, 16448250, 16728642, 982784, 4375295, 13827953, 13457919, 16757522, 4343295, 16728758, 5898228, 16448250, 16728642, 982784, 4375295, 13827953, 13457919, 16757522, 4343295, 16728758, 5898228]  # ColorDefaults
            n230 = event-data() -> ()  [unwired: 1 in, 6 out]
            n231 = local write "_Add"(FALSE ("_Refresh")) -> ()
            n232 = local read "_VisiblePlots"() -> (w274:bool[])
            n233 = local read "CalPointIDs"() -> (w277:sgl[])
            n234 = local read "SliderMax"() -> (w279:sgl[])
            n235 = local read "SliderMin"() -> (w278:sgl[])
            n236 = local read "Colors"() -> (w270:sgl[])
            n237 = local read "N Items"() -> (w263:u8)
            n238 = local read "_CalpointIDSelect"() -> (w276:u16)
            n239 = local read "_Slider Max"() -> (w281:sgl)
            n240 = local read "_Slider Min"() -> (w280:sgl)
            n241 = Increment(x=w263) -> (x+1=w264:u8)
            n242 = local read "N Items"() -> (w262:u8)
            n243 = Greater Than 0?(x=w264) -> (x > 0?=w265:bool)
            n244 = Index Array(array=w271, index=w264) -> (element=w269:u32)
            n245 = Select(t=T9."Enabled" ("Disabled"), s=w265, f=T9."Disabled and Grayed Out" ("Disabled")) -> (s? t:f=w267:T9)
            n246 = Insert Into Array(array=w270, index=w262, new element=w269) -> (w282:sgl[])
            n247 = Insert Into Array(array=w279, index=w262, new element=w281) -> (w283:sgl[])
            n248 = Insert Into Array(array=w278, index=w262, new element=w280) -> (w284:sgl[])
            n249 = Insert Into Array(array=w277, index=w262, new element=w276) -> (w285:sgl[])
            n250 = Replace Array Subset(array=w274, new element=TRUE ("new element/subarray"), index=w262) -> (w273:bool[])
            n251 = property on="_Delete" class="Bool (strict)"("DisabledEnum"=w267) -> ()  [unwired: 2 in, 2 out]
            n252 = property on="N Items" class="DigNum (strict)"("Val(Sgnl)"=w264) -> ()  [unwired: 2 in, 2 out]
            n253 = property on="Colors" class="Arr (strict)"("Val(Sgnl)"=w282) -> ()  [unwired: 2 in, 2 out]
            n254 = property on="SliderMax" class="Arr (strict)"("Val(Sgnl)"=w283) -> ()  [unwired: 2 in, 2 out]
            n255 = property on="SliderMin" class="Arr (strict)"("Val(Sgnl)"=w284) -> ()  [unwired: 2 in, 2 out]
            n256 = property on="CalPointIDs" class="Arr (strict)"("Val(Sgnl)"=w285) -> ()  [unwired: 2 in, 2 out]
            n257 = property on="_VisiblePlots" class="Arr (strict)"("Val(Sgnl)"=w273) -> ()  [unwired: 2 in, 2 out]
            n258 = property on="_Refresh" class="Bool (strict)"("Val(Sgnl)"=TRUE ("Value (Signaling)")) -> ()  [unwired: 2 in, 2 out]
          }
          event "_Up": Value Change {
            n259 = event-data() -> ()  [unwired: 1 in, 6 out]
            n260 = stacked-sequence {
              frame #0 {
                n261 = property on="_Table" class="MCListbox (strict)"() -> ("ItemNames"=w301:string[][])  [unwired: 2 in, 2 out]
                n262 = local read "_Table"() -> (w300:i32)
                n263 = local read "_VisiblePlots"() -> (w298:bool[])
                n264 = local read "CalPointIDs"() -> (w294:sgl[])
                n265 = Array Size(array=w301) -> (size(s)=w313:i32[])
                n266 = local read "SliderMax"() -> (w296:sgl[])
                n267 = local read "SliderMin"() -> (w295:sgl[])
                n268 = local read "Colors"() -> (w297:sgl[])
                n269 = Index Array(array=w313) -> (element=w312:i32)  [unwired: 1 in]
                n270 = Decrement(x=w312) -> (x-1=w315:i32)
                n271 = Decrement(x=w300) -> (x-1=w314:i32)
                n272 = Delete From Array(array=w297, index=w300) -> (deleted portion=w311:sgl, array with subset deleted=w306:sgl[])  [unwired: 1 in]
                n273 = Delete From Array(array=w296, index=w300) -> (deleted portion=w310:sgl, array with subset deleted=w305:sgl[])  [unwired: 1 in]
                n274 = Delete From Array(array=w295, index=w300) -> (deleted portion=w309:sgl, array with subset deleted=w307:sgl[])  [unwired: 1 in]
                n275 = Delete From Array(array=w294, index=w300) -> (deleted portion=w308:sgl, array with subset deleted=w304:sgl[])  [unwired: 1 in]
                n276 = Delete From Array(array=w298, index=w300) -> (deleted portion=w302:bool, array with subset deleted=w303:bool[])  [unwired: 1 in]
                n277 = In Range and Coerce(upper limit=w315, x=w314, lower limit=0) -> (coerced(x)=w299:i32)  [unwired: 1 out]
                n278 = Insert Into Array(array=w306, index=w299, new element=w311) -> (w289:sgl[])
                n279 = Insert Into Array(array=w305, index=w299, new element=w310) -> (w290:sgl[])
                n280 = Insert Into Array(array=w307, index=w299, new element=w309) -> (w291:sgl[])
                n281 = Insert Into Array(array=w304, index=w299, new element=w308) -> (w292:sgl[])
                n282 = Insert Into Array(array=w303, index=w299, new element=w302) -> (w293:bool[])
                n283 = local write "_Table"(w299) -> ()
                n284 = property on="Colors" class="Arr (strict)"("Val(Sgnl)"=w289) -> ()  [unwired: 2 in, 2 out]
                n285 = property on="SliderMax" class="Arr (strict)"("Val(Sgnl)"=w290) -> ()  [unwired: 2 in, 2 out]
                n286 = property on="SliderMin" class="Arr (strict)"("Val(Sgnl)"=w291) -> ()  [unwired: 2 in, 2 out]
                n287 = property on="CalPointIDs" class="Arr (strict)"("Val(Sgnl)"=w292) -> ()  [unwired: 2 in, 2 out]
                n288 = property on="_VisiblePlots" class="Arr (strict)"("Val(Sgnl)"=w293) -> ()  [unwired: 2 in, 2 out]
              }
              frame #1 {
                n289 = property on="_Chart" class="WFChart (strict)"("History Data"=T10 []) -> ()  [unwired: 2 in, 2 out]
              }
            }
            n290 = local write "_Up"(FALSE ("_Up")) -> ()
            n291 = property on="_Refresh" class="Bool (strict)"("Val(Sgnl)"=TRUE ("Value (Signaling)")) -> ()  [unwired: 2 in, 2 out]
          }
          event "_Down": Value Change {
            n292 = event-data() -> ()  [unwired: 1 in, 6 out]
            n293 = stacked-sequence {
              frame #0 {
                n294 = property on="_Table" class="MCListbox (strict)"() -> ("ItemNames"=w332:string[][])  [unwired: 2 in, 2 out]
                n295 = local read "_Table"() -> (w331:i32)
                n296 = local read "_VisiblePlots"() -> (w329:bool[])
                n297 = local read "CalPointIDs"() -> (w325:sgl[])
                n298 = Array Size(array=w332) -> (size(s)=w344:i32[])
                n299 = local read "SliderMax"() -> (w327:sgl[])
                n300 = local read "SliderMin"() -> (w326:sgl[])
                n301 = local read "Colors"() -> (w328:sgl[])
                n302 = Index Array(array=w344) -> (element=w343:i32)  [unwired: 1 in]
                n303 = Decrement(x=w343) -> (x-1=w346:i32)
                n304 = Increment(x=w331) -> (x+1=w345:i32)
                n305 = Delete From Array(array=w328, index=w331) -> (deleted portion=w342:sgl, array with subset deleted=w337:sgl[])  [unwired: 1 in]
                n306 = Delete From Array(array=w327, index=w331) -> (deleted portion=w341:sgl, array with subset deleted=w336:sgl[])  [unwired: 1 in]
                n307 = Delete From Array(array=w326, index=w331) -> (deleted portion=w340:sgl, array with subset deleted=w338:sgl[])  [unwired: 1 in]
                n308 = Delete From Array(array=w325, index=w331) -> (deleted portion=w339:sgl, array with subset deleted=w335:sgl[])  [unwired: 1 in]
                n309 = Delete From Array(array=w329, index=w331) -> (deleted portion=w333:bool, array with subset deleted=w334:bool[])  [unwired: 1 in]
                n310 = In Range and Coerce(upper limit=w346, x=w345, lower limit=0) -> (coerced(x)=w330:i32)  [unwired: 1 out]
                n311 = Insert Into Array(array=w337, index=w330, new element=w342) -> (w320:sgl[])
                n312 = Insert Into Array(array=w336, index=w330, new element=w341) -> (w321:sgl[])
                n313 = Insert Into Array(array=w338, index=w330, new element=w340) -> (w322:sgl[])
                n314 = Insert Into Array(array=w335, index=w330, new element=w339) -> (w323:sgl[])
                n315 = Insert Into Array(array=w334, index=w330, new element=w333) -> (w324:bool[])
                n316 = local write "_Table"(w330) -> ()
                n317 = property on="Colors" class="Arr (strict)"("Val(Sgnl)"=w320) -> ()  [unwired: 2 in, 2 out]
                n318 = property on="SliderMax" class="Arr (strict)"("Val(Sgnl)"=w321) -> ()  [unwired: 2 in, 2 out]
                n319 = property on="SliderMin" class="Arr (strict)"("Val(Sgnl)"=w322) -> ()  [unwired: 2 in, 2 out]
                n320 = property on="CalPointIDs" class="Arr (strict)"("Val(Sgnl)"=w323) -> ()  [unwired: 2 in, 2 out]
                n321 = property on="_VisiblePlots" class="Arr (strict)"("Val(Sgnl)"=w324) -> ()  [unwired: 2 in, 2 out]
              }
              frame #1 {
                n322 = property on="_Chart" class="WFChart (strict)"("History Data"=T10 []) -> ()  [unwired: 2 in, 2 out]
              }
            }
            n323 = local write "_Down"(FALSE ("_Up")) -> ()
            n324 = property on="_Refresh" class="Bool (strict)"("Val(Sgnl)"=TRUE ("Value (Signaling)")) -> ()  [unwired: 2 in, 2 out]
          }
          event "_Delete": Value Change {
            n325 = event-data() -> ()  [unwired: 1 in, 6 out]
            n326 = local write "_Delete"(FALSE ("_Refresh")) -> ()
            n327 = stacked-sequence {
              frame #0 {
                n328 = local read "Colors"() -> (w363:sgl[])
                n329 = local read "_Table"() -> (w359:i32)
                n330 = local read "_VisiblePlots"() -> (w360:bool[])
                n331 = local read "N Items"() -> (w352:u8)
                n332 = local read "CalPointIDs"() -> (w368:sgl[])
                n333 = local read "SliderMax"() -> (w362:sgl[])
                n334 = local read "SliderMin"() -> (w361:sgl[])
                n335 = Decrement(x=w352) -> (x-1=w351:u8)
                n336 = Delete From Array(array=w363, index=w359) -> (array with subset deleted=w367:sgl[])  [unwired: 1 in, 1 out]
                n337 = Delete From Array(array=w362, index=w359) -> (array with subset deleted=w366:sgl[])  [unwired: 1 in, 1 out]
                n338 = Delete From Array(array=w361, index=w359) -> (array with subset deleted=w365:sgl[])  [unwired: 1 in, 1 out]
                n339 = Delete From Array(array=w368, index=w359) -> (array with subset deleted=w364:sgl[])  [unwired: 1 in, 1 out]
                n340 = Replace Array Subset(array=w360, new element=FALSE ("new element/subarray"), index=w351) -> (w358:bool[])
                n341 = property on="N Items" class="DigNum (strict)"("Val(Sgnl)"=w351) -> ()  [unwired: 2 in, 2 out]
                n342 = property on="Colors" class="Arr (strict)"("Val(Sgnl)"=w367) -> ()  [unwired: 2 in, 2 out]
                n343 = property on="SliderMax" class="Arr (strict)"("Val(Sgnl)"=w366) -> ()  [unwired: 2 in, 2 out]
                n344 = property on="SliderMin" class="Arr (strict)"("Val(Sgnl)"=w365) -> ()  [unwired: 2 in, 2 out]
                n345 = property on="CalPointIDs" class="Arr (strict)"("Val(Sgnl)"=w364) -> ()  [unwired: 2 in, 2 out]
                n346 = property on="_VisiblePlots" class="Arr (strict)"("Val(Sgnl)"=w358) -> ()  [unwired: 2 in, 2 out]
                n347 = Greater Than 0?(x=w351) -> (x > 0?=w354:bool)
                n348 = Select(t=T9."Enabled" ("Disabled"), s=w354, f=T9."Disabled and Grayed Out" ("Disabled")) -> (s? t:f=w357:T9)
                n349 = property on="_Delete" class="Bool (strict)"("DisabledEnum"=w357) -> ()  [unwired: 2 in, 2 out]
              }
              frame #1 {
                n350 = property on="_Chart" class="WFChart (strict)"("History Data"=T10 []) -> ()  [unwired: 2 in, 2 out]
              }
            }
            n351 = property on="_Refresh" class="Bool (strict)"("Val(Sgnl)"=TRUE ("Value (Signaling)")) -> ()  [unwired: 2 in, 2 out]
          }
          event "_Default Colors": Value Change {
            n352 = event-data() -> ("NewVal"=w370:bool)  [unwired: 1 in, 5 out]
            n353 = case shown="True" w370 {
              frame False {
              }
              frame True {
                w371 = u32[] [483491, 16728642, 982784, 4375295, 13827953, 13457919, 16757522, 4343295, 16728758, 5898228, 0, 16728642, 982784, 4375295, 13827953, 13457919, 16757522, 4343295, 16728758, 5898228, 0, 16728642, 982784, 4375295, 13827953, 13457919, 16757522, 4343295, 16728758, 5898228, 0, 16728642, 982784, 4375295, 13827953, 13457919, 16757522, 4343295, 16728758, 5898228, 0, 16728642, 982784, 4375295, 13827953, 13457919, 16757522, 4343295, 16728758, 5898228, 0, 16728642, 982784, 4375295, 13827953, 13457919, 16757522, 4343295, 16728758, 5898228, 0, 16728642, 982784, 4375295, 13827953, 13457919, 16757522, 4343295, 16728758, 5898228, 0, 16728642, 982784, 4375295, 13827953, 13457919, 16757522, 4343295, 16728758, 5898228, 0, 16728642, 982784, 4375295, 13827953, 13457919, 16757522, 4343295, 16728758, 5898228, 0, 16728642, 982784, 4375295, 13827953, 13457919, 16757522, 4343295, 16728758, 5898228]  # ColorDefaults
                n354 = property on="Colors" class="Arr (strict)"("Val(Sgnl)"=w371) -> ()  [unwired: 2 in, 2 out]
              }
            }
          }
        }
      }
    }
  }
